vi "Test.vi"() -> ()   [LabVIEW 2018]
panel:
  out "成功？":bool
  out "Time has Elapsed":bool caption="超时？"
  in  "超时时间MS":dbl
  in  "设定时间MS":dbl
  in  "变量":dbl
  in  "设定值上限":dbl
  in  "设定值下限":dbl
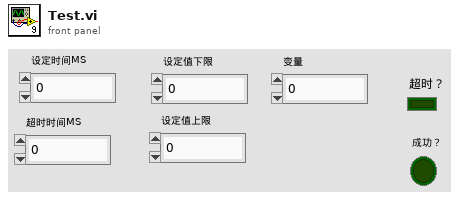
[diagram p1: front panel]
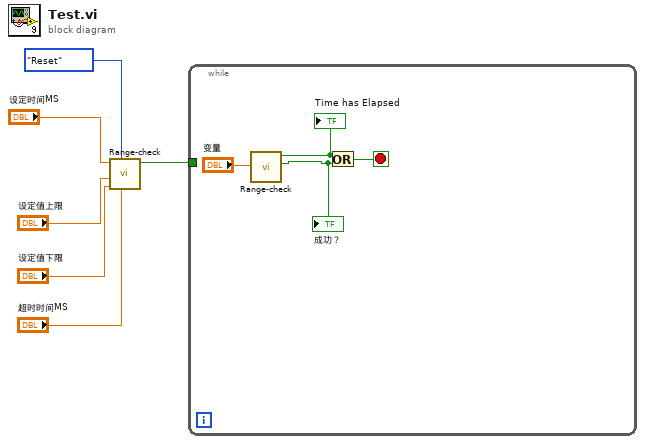
[diagram p0: block diagram]
diagram:
  n1 = call "Range-check.vi"("超时时间（Ms）"="超时时间MS", "枚举"=enum16{"Reset", "usage"}."Reset", "设定值下限"="设定值下限", "设定值上限"="设定值上限", "设定时间MS"="设定时间MS") -> ("Time has Elapsed"=w2:bool)  [unwired: 5 in, 1 out]
  n2 = while {
    tunnel: w2 -> [_]
    stop <- w7 stop-if-true
    n3 = call "Range-check.vi"("变量"="变量") -> ("成功？"=w8:bool, "Time has Elapsed"=w9:bool)  [unwired: 9 in]
    "Time has Elapsed" <- w9
    "成功？" <- w8
    n4 = Or(x=w9, y=w8) -> (x .or. y?=w7:bool)
  }
